vi "GetSetInteger.vi"(7 "Set?":bool, 8 "error in (no error)":errorcluster, 9 "Value in":i64, 10 "Name":string, 11 "Camera in":refnum<class "Camera.lvclass">) -> (0 "error out":errorcluster, 1 "Value out":i64)   [LabVIEW 2020, in "Camera.lvclass"]
uses:
  Camera.lvclass
  Camera.lvclass/Camera.ctl
  bin/gindustrialcam_32-1.dll
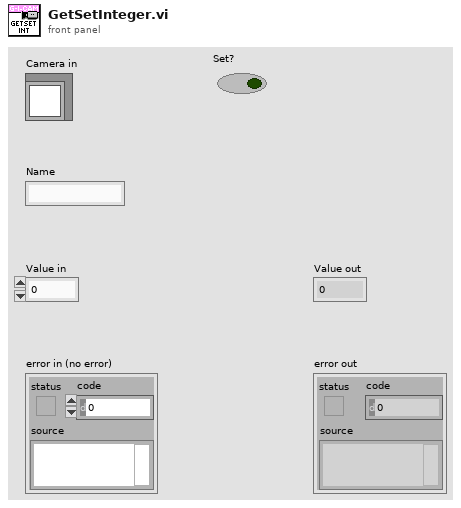
[diagram p1: front panel]
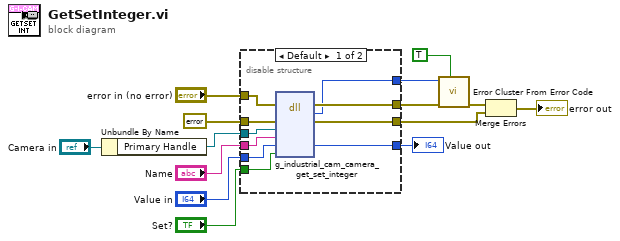
[diagram p0: block diagram]
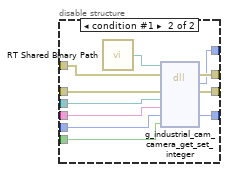
[diagram p2: hidden frame]
diagram:
  n1 = Unbundle By Name("Camera in") -> ("Primary Handle"=w3:refnum<data-value>)
  n2 = disable-structure shown="Default" {
    disable-tunnel: [w24 w35] -> w14
    disable-tunnel: [w23 w34] -> w13
    disable-tunnel: [w22 w33] -> w11
    disable-tunnel: errorcluster {"status"=FALSE, "code"=0, "source"=""} ("error constant") -> [w21 w32]
    disable-tunnel: "error in (no error)" -> [w20 w31]
    disable-tunnel: "Name" -> [w19 w30]
    disable-tunnel: "Set?" -> [w18 w29]
    disable-tunnel: w3 -> [w17 w28]
    disable-tunnel: "Value in" -> [w16 w27]
    disable-tunnel: [w15 w26] -> w1
    frame condition #0 (active) {
      n3 = dll-call lib="C:/serenial/lib/g-industrial-camera/LabVIEW/g_industrial_cam/bin/gindustrialcam_*-1.*" fn="g_industrial_cam_camera_get_set_integer"(error in=w20, "err"=w21, "edvr"=w17, "name"=w19, "value"=w16, "set"=w18) -> (error out=w24:errorcluster, "Mg_Error"=w23:i32, "err"=w22:errorcluster, "value"=w15:i64)  [unwired: 5 in, 1 out]
    }
    frame condition #1 {
      n4 = call "RT Shared Binary Path.vi"() -> ("Path"=w25:path)
      n5 = dll-call lib="C:/serenial/lib/g-industrial-camera/LabVIEW/g_industrial_cam/bin/gindustrialcam_*-1.*" fn="g_industrial_cam_camera_get_set_integer"(path in=w25, error in=w31, "err"=w32, "edvr"=w28, "name"=w30, "value"=w27, "set"=w29) -> (error out=w35:errorcluster, "Mg_Error"=w34:i32, "err"=w33:errorcluster, "value"=w26:i64)  [unwired: 4 in, 1 out]
    }
  }
  "Value out" <- w1
  n6 = call <vilib>:"Error Cluster From Error Code.vi"("show call chain? (False)"=TRUE, "error in (no error)"=w14, "error code (0)"=w13) -> ("error out"=w12:errorcluster)  [unwired: 6 in]
  n7 = Merge Errors(w12, w11) -> (→"error out":errorcluster)
